vi "Trigger Channel.vi"(8 "error in (no error)":errorcluster, 11 "Node Ptr":T1 format="%.0x") -> (0 "error out":errorcluster)   [LabVIEW 2020, in "Instrument Addon System Explorer.lvlib"]
uses:
  Instrument Addon System Explorer.lvlib
  <vilib>/NI VeriStand/Custom Device API/Custom Device API.lvlib
  <vilib>/NI VeriStand/UI Controls/Single Node Browser/NI_VS UI Single Node Browser.lvlib
  NationalInstruments.VeriStand.SystemStorage
  Addon Shared/Types/FG Control.ctl
  Addon Shared/Instrument Addon Shared.lvlib
  Addon Shared/SubVIs/Constants.vi
  <vilib>/NI VeriStand/Custom Device API/Custom Device Item Ref.ctl
  NationalInstruments.VeriStand.SystemStorageUI
panel:
  in  "Header 2":cluster{"Section Name":string}={"Section Name"="External Trigger Settings"}
  in  "Channel":refnum<k24>(container) caption="Value"
  in  "Use Channel?":bool
  in  "SHDocVw.IWebBrowser":refnum<k7>(container)
  in  "Header":cluster{"Section Name":string}={"Section Name"="Trigger Settings"}
  in  "Description":string
  out "Name":string
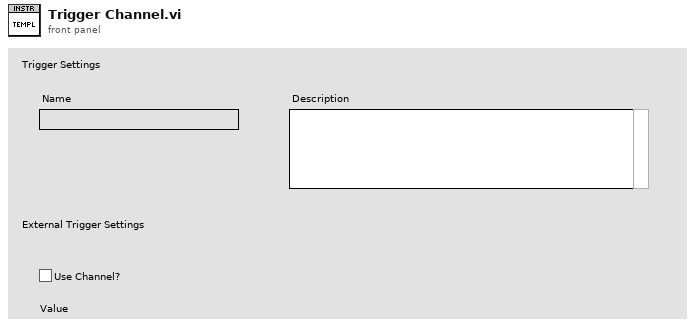
[diagram p1: front panel]
types:
  T1 = typedef "Custom Device API.lvlib/Custom Device Item Ref.ctl" = u64
  T2 = typedef "Instrument Addon Shared.lvlib/FG Control.ctl" = enum16{"Get", "Set"}
  T3 = typedef "Instrument Addon Shared.lvlib/Trigger Parameters.ctl" = cluster{"Use Channel":bool, "Channel Path":string}
  T4 = typedef "Custom Device API.lvlib/Custom Device Item Info.ctl" = cluster{"Name":string, "Is Channel":bool, "GUID":string, "Is Waveform":bool}
  T5 = typedef "Custom Device API.lvlib/Custom Device Commands.ctl" = enum16{"Default", "Item renamed", "Shutdown", "Dynamic button pressed"}
  T6 = typedef "NI_VS UI Single Node Browser.lvlib/Node Ref.ctl" = refnum<k24>
  T7 = typedef "Custom Device API.lvlib/Custom Device Pointer.ctl" = refnum<k24>
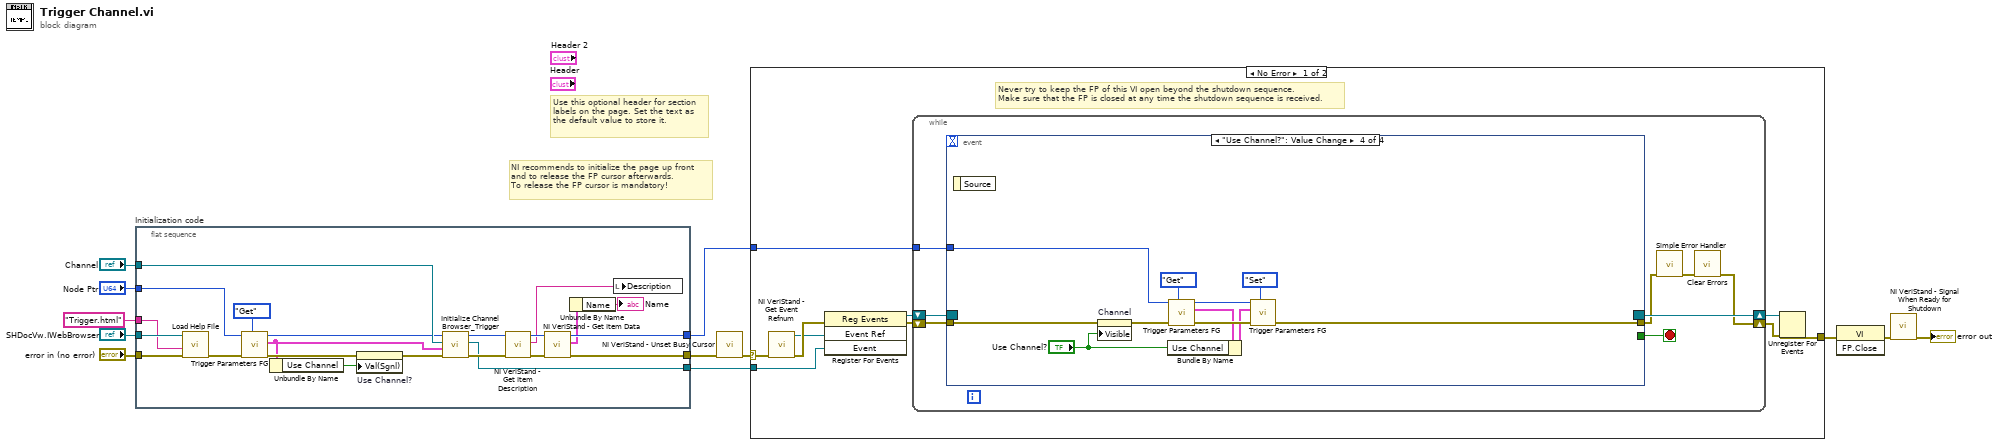
[diagram p0: block diagram]
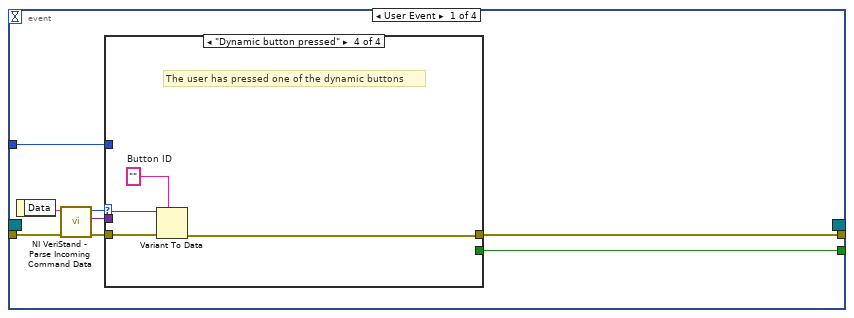
[diagram p2: hidden frame]
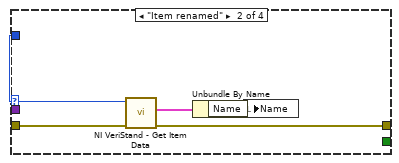
[diagram p4: hidden frame]
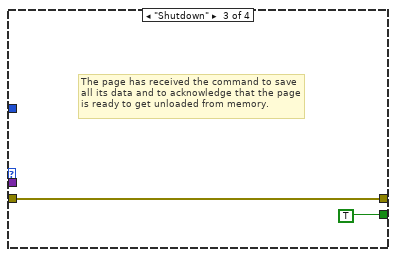
[diagram p5: hidden frame]
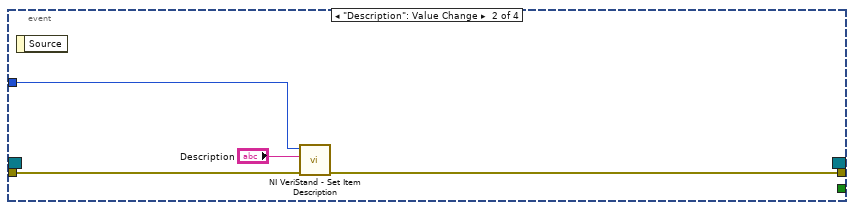
[diagram p6: hidden frame]
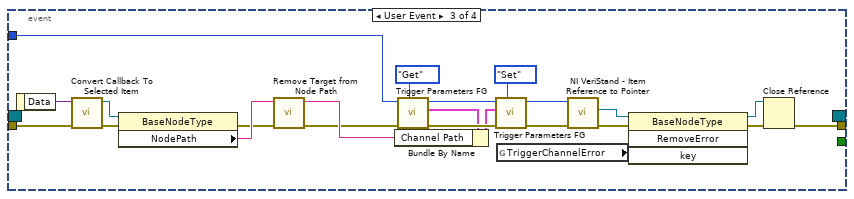
[diagram p7: hidden frame]
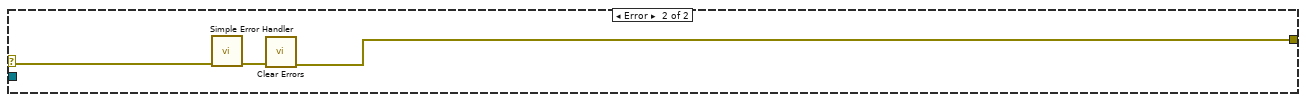
[diagram p8: hidden frame]
diagram:
  # "Use this optional header for section labels on the page. Set the text as the default value to store it."
  # "NI recommends to initialize the page up front\nand to release the FP cursor afterwards.\nTo release the FP cursor is mandatory!"
  n1 = flat-sequence "Initialization code" {
    tunnel: "error in (no error)" -> [w27]
    tunnel: "Node Ptr" -> [w18]
    tunnel: [w29] -> w8
    tunnel: [w34] -> w5
    tunnel: "SHDocVw.IWebBrowser" -> [w26]
    tunnel: "Trigger.html" ("HTML File") -> [w25]
    tunnel: "Channel" -> [w22]
    tunnel: [w21] -> w1
    frame #0 {
      n2 = call "Load Help File.vi"("error in (no error)"=w27, "HTML File to Load"=w25, "SHDocVw.IWebBrowser2"=w26) -> ("error out"=w19:errorcluster)  [unwired: 8 in]
      n3 = call "Trigger Parameters FG.vi"("Action"=FG_Control."Get", "error in (no error)"=w19, "Item Ref in"=w18) -> ("error out"=w16:errorcluster, "Trigger Parameters"=w13:T3, "Item Ref out"=w17:T1)  [unwired: 6 in]
      n4 = Unbundle By Name(w13) -> ("Use Channel"=w14:bool)
      n5 = property on="Use Channel?" class="Bool (strict)"(error in=w16, "Val(Sgnl)"=w14) -> (error out=w15:errorcluster)  [unwired: 1 in, 1 out]
      n6 = call "Initialize Channel Browser_Trigger.vi"("error in (no error)"=w15, "Trigger Parameters"=w13, ".NET Refnum in"=w22, "Item Ref in"=w17) -> ("error out"=w24:errorcluster, "Event"=w21:refnum<user-event>, "Item Ref out"=w23:T1)  [unwired: 5 in]
      n7 = call <vilib>:"NI VeriStand - Get Item Description.vi"("error in (no error)"=w24, "Item Ref in"=w23) -> ("error out"=w31:errorcluster, "Description"=w32:string, "Item Ref out"=w33:T1)  [unwired: 7 out]
      n8 = call <vilib>:"NI VeriStand - Get Item Data.vi"("error in (no error)"=w31, "Item Ref in"=w33) -> ("error out"=w29:errorcluster, "Item Info"=w30:T4, "Item Ref out"=w34:T1)  [unwired: 7 out]
      n9 = Unbundle By Name(w30) -> ("Name"=→"Name":string)
      n10 = local write "Description"(w32) -> ()
    }
  }
  n11 = call <vilib>:"NI VeriStand - Unset Busy Cursor.vi"("error in (no error)"=w8) -> ("error out"=w7:errorcluster)  [unwired: 10 out]
  n12 = case shown="No Error" w7 {
    selector: w7 -> [w36 w113]
    tunnel: [w41 w111] -> w12
    tunnel: w5 -> [w37 _]
    tunnel: w1 -> [w35 _]
    frame No Error {
      # "Never try to keep the FP of this VI open beyond the shutdown sequence.\nMake sure that the FP is closed at any time the shutdown sequence is received."
      n13 = call <vilib>:"NI VeriStand - Get Event Refnum.vi"("error in (no error)"=w36) -> ("error out"=w44:errorcluster, "Event Ref"=w40:refnum<user-event>)  [unwired: 9 out]
      n14 = register-events(error in=w44, w40, w35) -> (reference out=w38:refnum<event-registration>, error out=w39:errorcluster)  [unwired: 1 in]
      n15 = while {
        tunnel: w37 -> [w48]
        shift-right: [w45] -> w42
        shift-left: w39 -> [w51]
        shift-right: [w52] -> w43
        shift-left: w38 -> [w50]
        stop <- w49 stop-if-true
        n16 = event shown="[3] \"Use Channel?\": Value Change" {
          selector: w50 -> [_ _ _ _]
          dyn-events: [_ _ _ _] -> w52
          timeout: _ -> [_ _ _ _]
          tunnel: w51 -> [w60 w75 w80 w105]
          tunnel: [w56 _ _ _] -> w49
          tunnel: [w55 w74 w81 w100] -> w47
          tunnel: w48 -> [w54 w76 w78 w101]
          event User Event {
            n17 = event-data() -> ("Data"=w59:string)  [unwired: 1 out]
            n18 = call <vilib>:"NI VeriStand - Parse Incoming Command Data.vi"("error in (no error)"=w60, "Incoming data"=w59) -> ("error out"=w58:errorcluster, "Outgoing data"=w53:variant, "Action"=w57:T5)  [unwired: 7 out]
            n19 = case shown="\"Dynamic button pressed\"" w57 {
              tunnel: w58 -> [w61 w66 w67 w72]
              tunnel: [_ _ TRUE _] -> w56
              tunnel: [w61 w63 w67 w69] -> w55
              tunnel: w54 -> [_ w65 _ _]
              tunnel: w53 -> [_ _ _ w71]
              frame "Default", Default {
              }
              frame "Item renamed" {
                n20 = call <vilib>:"NI VeriStand - Get Item Data.vi"("error in (no error)"=w66, "Item Ref in"=w65) -> ("error out"=w63:errorcluster, "Item Info"=w64:T4)  [unwired: 8 out]
                n21 = Unbundle By Name(w64) -> ("Name"=w62:string)
                n22 = local write "Name"(w62) -> ()
              }
              frame "Shutdown" {
                # "The page has received the command to save all its data and to acknowledge that the page is ready to get unloaded from memory."
              }
              frame "Dynamic button pressed" {
                w70 = ""  # Button ID
                # "The user has pressed one of the dynamic buttons"
                n23 = Variant To Data(error in=w72, type=w70, Variant=w71) -> (error out=w69:errorcluster)  [unwired: 1 out]
              }
            }
          }
          event "Description": Value Change {
            n24 = event-data() -> ()  [unwired: 2 out]
            n25 = call <vilib>:"NI VeriStand - Set Item Description.vi"("error in (no error)"=w75, "Description"="Description", "Item Ref in"=w76) -> ("error out"=w74:errorcluster)  [unwired: 8 out]
          }
          event User Event {
            n26 = event-data() -> ("Data"=w79:variant)  [unwired: 1 out]
            n27 = call <vilib>:"Convert Callback To Selected Item.vi"("error in"=w80, "Data"=w79) -> ("error out"=w83:errorcluster, "Selected Item"=w82:T6)  [unwired: 8 in]
            n28 = property class="BaseNodeType"(reference=w82, error in=w83) -> (error out=w89:errorcluster, "NodePath"=w90:string)  [unwired: 1 out]
            n29 = call "Remove Target from Node Path.vi"("error in (no error)"=w89, "NodePath"=w90) -> ("error out"=w91:errorcluster, "PathArrayToString"=w92:string)  [unwired: 8 in]
            n30 = call "Trigger Parameters FG.vi"("Action"=FG_Control."Get", "error in (no error)"=w91, "Item Ref in"=w78) -> ("error out"=w88:errorcluster, "Trigger Parameters"=w86:T3, "Item Ref out"=w87:T1)  [unwired: 6 in]
            n31 = Bundle By Name(cluster=w86, "Channel Path"=w92) -> (w77:T3)
            n32 = call "Trigger Parameters FG.vi"("Action"=FG_Control."Set", "error in (no error)"=w88, "Trigger Parameters"=w77, "Item Ref in"=w87) -> ("error out"=w97:errorcluster, "Item Ref out"=w98:T1)  [unwired: 5 in, 1 out]
            n33 = global read "Constants.vi" "TriggerChannelError"() -> (w99:string)
            n34 = call <vilib>:"NI VeriStand - Item Reference to Pointer.vi"("error in (no error)"=w97, "Item Ref in"=w98) -> ("error out"=w95:errorcluster, "Node Pointer"=w96:T7)  [unwired: 6 in, 2 out]
            n35 = invoke class="BaseNodeType" method="RemoveError"(reference=w96, error in=w95, "key"=w99) -> (reference out=w93:T7, error out=w94:errorcluster)  [unwired: 1 in, 2 out]
            n36 = Close Reference(reference=w93, error in (no error)=w94) -> (error out=w81:errorcluster)
          }
          event "Use Channel?": Value Change {
            n37 = event-data() -> ()  [unwired: 2 out]
            n38 = property on="Channel" class="AXCont"(error in=w105, "Visible"="Use Channel?") -> (error out=w104:errorcluster)  [unwired: 1 in, 1 out]
            n39 = call "Trigger Parameters FG.vi"("Action"=FG_Control."Get", "error in (no error)"=w104, "Item Ref in"=w101) -> ("error out"=w110:errorcluster, "Trigger Parameters"=w108:T3, "Item Ref out"=w109:T1)  [unwired: 6 in]
            n40 = Bundle By Name(cluster=w108, "Use Channel"="Use Channel?") -> (w106:T3)
            n41 = call "Trigger Parameters FG.vi"("Action"=FG_Control."Set", "error in (no error)"=w110, "Trigger Parameters"=w106, "Item Ref in"=w109) -> ("error out"=w100:errorcluster)  [unwired: 5 in, 2 out]
          }
        }
        n42 = call <vilib>:"Simple Error Handler.vi"("error in (no error)"=w47) -> ("error out"=w46:errorcluster)  [unwired: 1 in, 7 out]
        n43 = call <vilib>:"Clear Errors.vi"("error in (no error)"=w46) -> ("error out"=w45:errorcluster)  [unwired: 1 in, 5 out]
      }
      n44 = Unregister For Events(event registration refnum=w43, error in=w42) -> (error out=w41:errorcluster)
    }
    frame Error {
      n45 = call <vilib>:"Simple Error Handler.vi"("error in (no error)"=w113) -> ("error out"=w112:errorcluster)  [unwired: 1 in, 7 out]
      n46 = call <vilib>:"Clear Errors.vi"("error in (no error)"=w112) -> ("error out"=w111:errorcluster)  [unwired: 1 in, 5 out]
    }
  }
  n47 = invoke class="VI" method="FP.Close"(error in=w12) -> (error out=w11:errorcluster)  [unwired: 2 in, 2 out]
  n48 = call <vilib>:"NI VeriStand - Signal When Ready for Shutdown.vi"("error in (no error)"=w11) -> ("error out"=→"error out":errorcluster)  [unwired: 10 out]
